vi "Build Method Not Found Response.vi"(8 "error in":errorcluster, 11 "message json":string) -> (0 "error out":errorcluster, 3 "response":string)   [LabVIEW 2020, in "MCP Server.lvlib"]
doc: "Builds the answer to a JSON-RPC message whose method is not implemented.\n\nIf the message has a top-level id item (a request), response is a JSON-RPC error with code -32601, the message Method not found: followed by the method name, and the id of the request.\nIf the message has no top-level id item (a notification), response is an empty string, because a notification must never be answered.\n\nAn unknown method is a normal protocol answer, so no error is generated. error in is passed through unchanged."
uses:
  MCP Server.lvlib
  8e201dea-3a69-4711-8432-5aeeaeb0d043.vi
  <vilib>/JDP Science/JSONtext/Next JSON Value.vi
  <vilib>/JDP Science/JSONtext/String Subset.vi
  <vilib>/JDP Science/JSONtext/Parsing/Advance past next JSON Value (inlined COPY).vi
  <vilib>/JDP Science/JSONtext/Parsing/Advance past whitespace.vi
  <vilib>/JDP Science/JSONtext/Parsing/Advance past String.vi
  <vilib>/JDP Science/JSONtext/Parsing/Advance past Number.vi
  <vilib>/JDP Science/JSONtext/Parsing/Advance past Line Ending.vi
  <vilib>/JDP Science/JSONtext/Parsing/Parse Full Path or Item Name.vi
  <vilib>/JDP Science/JSONtext/Parsing/Advance past Array.vi
  <vilib>/JDP Science/JSONtext/Parsing/Advance past Object.vi
  <vilib>/JDP Science/JSONtext/support/Error Cluster From Code.vi
  <vilib>/JDP Science/JSONtext/Offset/Find Item Locations by Path.vi
  <vilib>/JDP Science/JSONtext/JSON text to Variant.vi
  <vilib>/JDP Science/JSONtext/LVClass Serializer/JSONtext LVClass Serializer.lvclass
  <vilib>/JDP Science/JSONtext/JSONtext.lvlib
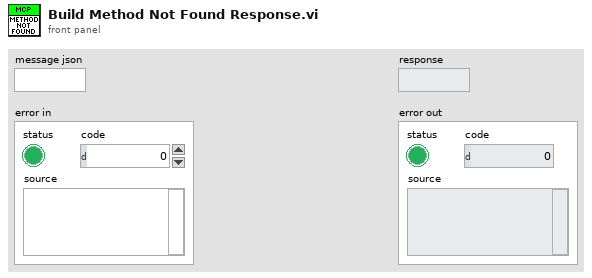
[diagram p1: front panel]
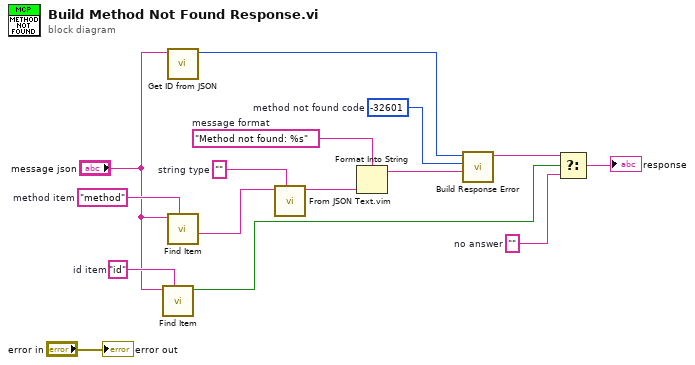
[diagram p0: block diagram]
diagram:
  w3 = ""  # no answer
  w7 = -32601  # method not found code
  w10 = "id"  # id item
  w11 = "Method not found: %s"  # message format
  w13 = ""  # string type
  w15 = "method"  # method item
  n1 = call <vilib>:"Find Item.vi"("$Path or Item Name"=w10, "JSON"="message json") -> ("Found"=w4:bool)  [unwired: 6 in, 3 out]
  n2 = call "Get ID from JSON.vi"("message json"="message json") -> ("Data out"=w8:i32)  [unwired: 10 in]
  n3 = call <vilib>:"Find Item.vi"("$Path or Item Name"=w15, "JSON"="message json") -> ("<JSON>"=w14:string)  [unwired: 6 in, 3 out]
  n4 = call "From JSON Text.vim"("Data Type and Default Value"=w13, "JSON"=w14) -> ("Data out"=w12:string)  [unwired: 8 in, 1 out]
  n5 = Format Into String(format string=w11, w12) -> (resulting string=w6:string)  [unwired: 2 in, 1 out]
  n6 = call "Build Response Error.vi"("message"=w6, "code"=w7, "message id in"=w8) -> ("MCP message out"=w5:string)  [unwired: 7 in, 1 out]
  n7 = Select(t=w5, s=w4, f=w3) -> (s? t:f=→"response":string)
  "error out" <- "error in"
